vi "Test All Instruments.vi"() -> ()   [LabVIEW 2026]
uses:
  Typedefs/Chiller Action.ctl
panel:
  out "XY Graph":cluster{dbl[], dbl[]}(graph)
  out "DAQ Temp (C)":dbl
  out "Chiller Temp (C)":dbl
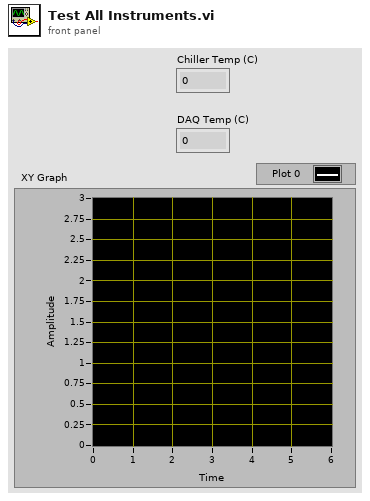
[diagram p1: front panel]
types:
  T1 = typedef "Chiller Action.ctl" = enum16{"Init", "Set Setpoint", "Step", "Read"}
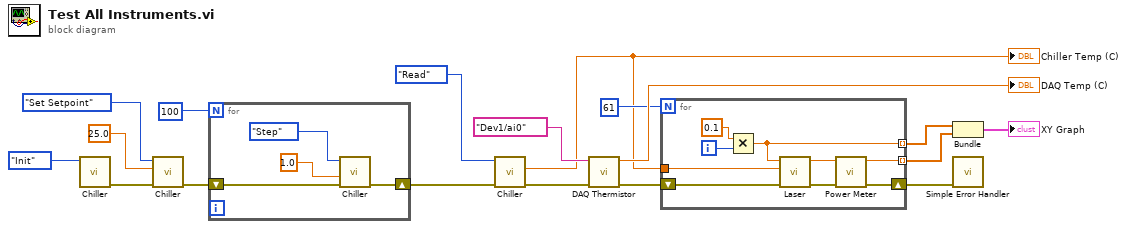
[diagram p0: block diagram]
diagram:
  n1 = call "Chiller.vi"("Action"=Chiller_Action."Init") -> ("error out"=w14:errorcluster)  [unwired: 6 in, 2 out]
  n2 = call "Chiller.vi"("error in (no error)"=w14, "Setpoint (C)"=25.0, "Action"=Chiller_Action."Set Setpoint") -> ("error out"=w13:errorcluster)  [unwired: 4 in, 2 out]
  n3 = for {
    N: 100 -> [_]
    shift-right: [w19] -> w12
    shift-left: w13 -> [w20]
    n4 = call "Chiller.vi"("error in (no error)"=w20, "dt (s)"=1.0, "Action"=Chiller_Action."Step") -> ("error out"=w19:errorcluster)  [unwired: 4 in, 2 out]
  }
  n5 = call "Chiller.vi"("error in (no error)"=w12, "Action"=Chiller_Action."Read") -> ("error out"=w6:errorcluster, "Temp (C)"=w7:dbl)  [unwired: 5 in, 1 out]
  "Chiller Temp (C)" <- w7
  n6 = call "DAQ Thermistor.vi"("error in (no error)"=w6, "DAQmx Physical Channel"=tag "Dev1/ai0") -> ("error out"=w5:errorcluster, "Temp (C)"=→"DAQ Temp (C)":dbl)  [unwired: 7 in, 1 out]
  n7 = for {
    N: 61 -> [_]
    tunnel: w7 -> [w29]
    shift-right: [w26] -> w4
    shift-left: w5 -> [w28]
    tunnel: [w24] -> w3 mode=indexing
    tunnel: [w23] -> w2 mode=indexing
    i -> [w31]
    n8 = Multiply(x=0.1, y=w31) -> (x*y=w24:dbl)
    n9 = call "Laser.vi"("error in (no error)"=w28, "Temp (C)"=w29, "Current (A)"=w24) -> ("error out"=w27:errorcluster, "Power (W)"=w25:dbl)  [unwired: 6 in, 1 out]
    n10 = call "Power Meter.vi"("error in (no error)"=w27, "True Power (W)"=w25) -> ("error out"=w26:errorcluster, "Reading (W)"=w23:dbl)  [unwired: 8 in]
  }
  n11 = Bundle(w3, w2) -> (→"XY Graph":cluster{dbl[], dbl[]})  [unwired: 1 in]
  n12 = call <vilib>:"Simple Error Handler.vi"("error in (no error)"=w4) -> ()  [unwired: 4 in, 5 out]
